vi "PicoScope2000aExampleBlockMSO.vi"() -> ()   [LabVIEW 2010]
doc: "ps2000a API Block Capture example"
uses:
  shared/PicoBuffers.ctl
  <vilib>/Waveform/DWDTOps.llb/DWDT Analog to Digital.vi
  shared/Buffer and Transfer Settings.ctl
  shared/Acquisition Settings.ctl
  PicoScope2000aLib/PicoScope2000aAnalogChannelSettings.ctl
  PicoScope2000aLib/PicoScope2000aDigitalChannelSettings.ctl
panel:
  out "Properties Panel":T1 {"Max Total Capture Time Available (sec)" format="%.3p"; "Sample Frequency" format="%.3p"; "Sample Internal" format="%.3p"; "Max Samples Available" format="%.3p"; "Total Capture Time (sec)" format="%.3p"}
  in  "Port 0 Settings":T2={"Enabled"=FALSE, "Logic Level"=9830} {"Logic Level" items=["1.5V TTL"=9830, "2.5V CMOS"=16383]}
  in  "Channel A Settings":T3={"Enabled"=TRUE, "Coupling"=1, "Range"=6, "Analogue Offset"=0.0} {"Analogue Offset" format="%#_6p"; "Range" items=["20 mV"=1, "50 mV"=2, "100 mV"=3, "200 mV"=4, "500 mV"=5, "1 V"=6, "2 V"=7, "5 V"=8, "10 V"=9, "20 V"=10]; "Coupling" items=["AC", "DC"]}
  out "Device Info":T4={"Driver Version"="2.1.104.3324", "USB Version"="2.0", "Hardware"="1", "Variant"="2206A", "Batch and Serial"="CV676/049", "Cal Date"="19Sep17", "Kernel Version"="1.0", "Digital HW Version"="1", "Analogue HW Version"="1", "Firmware 1"="1.3.3.0", "Firmware 2"="0.5.47.0", "MSO"=FALSE, "Number of Channels"=2}
  out "overflow":i16 format="%06b"
  in  "Apply Settings":bool
  in  "Trigger Settings":T5={"Trigger Enabled"=FALSE, "Trigger Source"=enum."Channel A", "Trigger Threshold (volts)"=0.0, "Trigger Direction"=2, "Trigger Delay (samples)"=0, "Auto Trigger Time (ms)"=1000} {"Trigger Direction" items=["Rising"=2, "Falling"=3]}
  out "error out":errorcluster
  in  "Data file":path=path "PicoScope2000aExampleBlock ChA Data"
  in  "Buffer and Transfer Settings":T6={"startIndex"=0, "Samples"=32000, "Down Sample Ratio"=1, "Down-Sample Mode"=0} {"Down-Sample Mode" items=["RAW none"=2147483648, "None"=0, "Aggregate"=1, "Decimate"=2, "Average"=4]; "Down Sample Ratio" step=1; "Samples" format="%_6p"}
  in  "Acquisition Settings":T7={"preTriggerSamples"=0, "postTriggerSamples"=32000, "timebase"=5} {"postTriggerSamples" format="%_6p"; "preTriggerSamples" format="%_6p"}
  out "Port 0":digitalwaveform(graph)={"t0"=timestamp(0 s since 1904-01-01), "dt"=8e-09, "Y"={"transitions"=[], "data"=[]}}
  in  "stop":bool
  out "Analog Channels":cluster{i32, sgl, "Data":dbl[]}[](graph)
  in  "Serial Number":string
  in  "Use Serial Number":bool
  in  "error in (no error)":errorcluster
  # "Bit 0 = ChA"
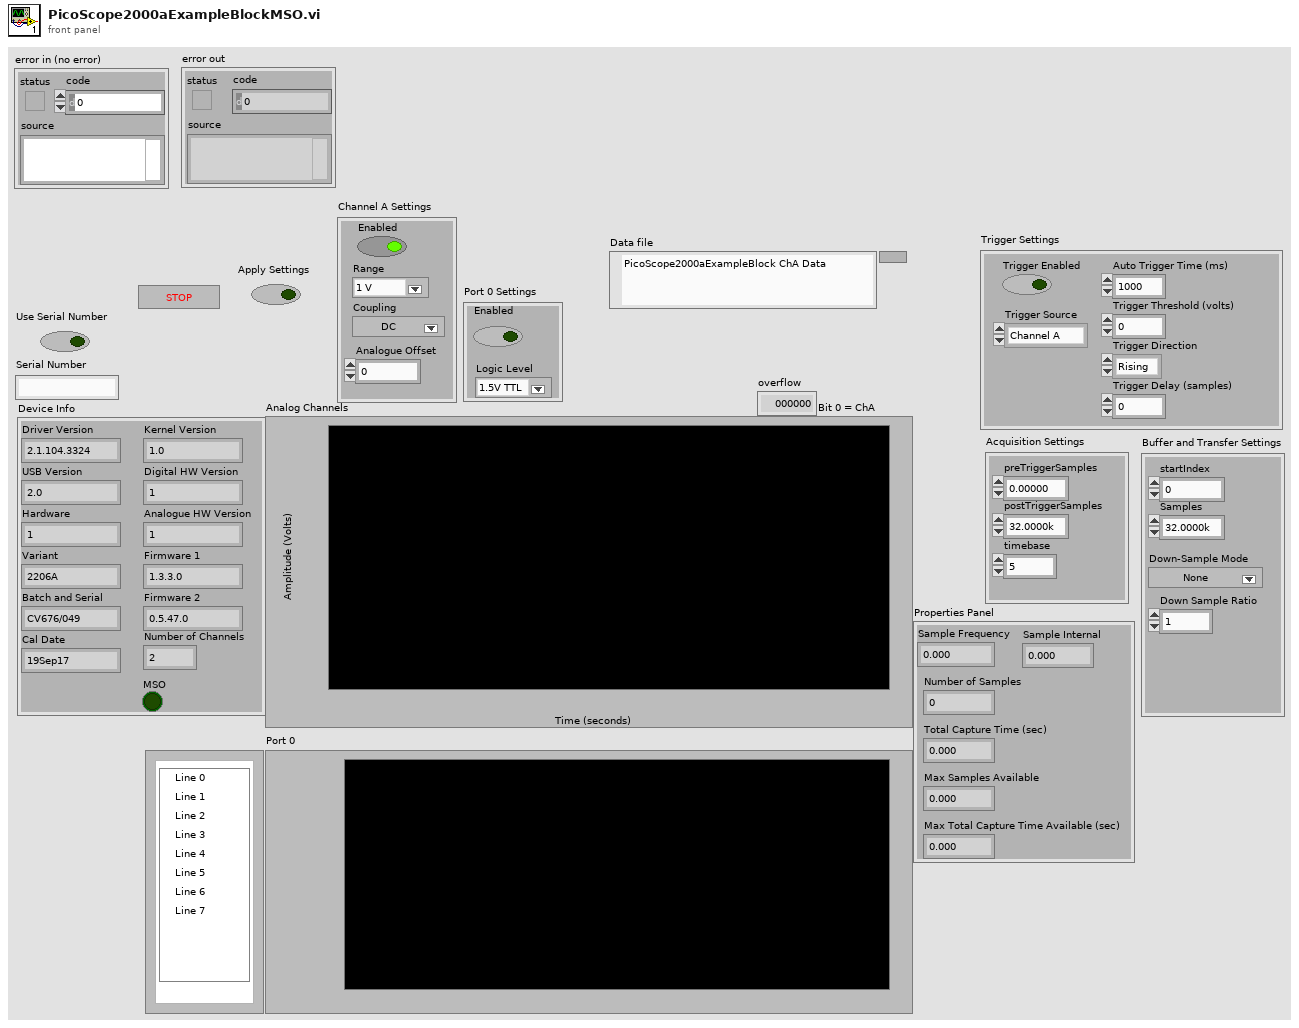
[diagram p1: front panel]
types:
  T1 = cluster{"Sample Frequency":sgl, "Sample Internal":sgl, "Max Samples Available":i32, "Number of Samples":u32, "Total Capture Time (sec) ":sgl, "Max Total Capture Time Available (sec)":sgl}
  T2 = typedef "PicoScope2000aDigitalChannelSettings.ctl" = cluster{"Enabled":bool, "Logic Level":i16}
  T3 = typedef "PicoScope2000aAnalogChannelSettings.ctl" = cluster{"Enabled":bool, "Coupling":i16, "Range":u16, "Analogue Offset":sgl}
  T4 = cluster{"Driver Version":string, "USB Version":string, "Hardware":string, "Variant":string, "Batch and Serial":string, "Cal Date":string, "Kernel Version":string, "Digital HW Version":string, "Analogue HW Version":string, "Firmware 1":string, "Firmware 2":string, "MSO":bool, "Number of Channels":i16}
  T5 = cluster{"Trigger Enabled":bool, "Trigger Source":enum16{"Channel A", "Channel B", "Channel C", "Channel D", "Ext."}, "Trigger Threshold (volts)":dbl, "Trigger Direction":u16, "Trigger Delay (samples)":u32, "Auto Trigger Time (ms)":i16}
  T6 = typedef "Buffer and Transfer Settings.ctl" = cluster{"startIndex":u64, "Samples":u64, "Down Sample Ratio":u64, "Down-Sample Mode":u32}
  T7 = typedef "Acquisition Settings.ctl" = cluster{"preTriggerSamples":u64, "postTriggerSamples":u64, "timebase":u32}
  T8 = enum16{"open", "open or create", "create or replace", "create", "open (read-only)"}
  T9 = typedef "PicoBuffers.ctl" = cluster{"Max Buffer Pointers":u64[][][], "Min Buffer Pointers":u64[][][], "StreamingDataInfo":cluster{"Channel":u32, "Down-Sample Mode":u32, "PICO_DATA_TYPE":enum32{"PICO_INT8_T", "PICO_INT16_T", "PICO_INT32_T", "PICO_UINT32_T", "PICO_INT64_T", ""}, "Samples":i32, "bufferIndex":u64, "startIndex":i32, "overflow":i16}[][]}
  T10 = cluster{"Channel A Buffer":i16[], "Channel B Buffer":i16[], "Channel C Buffer":i16[], "Channel D Buffer":i16[], "Channel E Buffer":i16[], "Channel F Buffer":i16[], "Channel G Buffer":i16[], "Channel H Buffer":i16[], "Port 0 Buffer":i16[], "Port 1 Buffer":i16[]}[]
  T11 = cluster{"Channel A Buffer":i16[], "Channel B Buffer":i16[], "Channel C Buffer":i16[], "Channel D Buffer":i16[], "Channel E Buffer":i16[], "Channel F Buffer":i16[], "Channel G Buffer":i16[], "Channel H Buffer":i16[], "Port 0 Buffer":i16[], "Port 1 Buffer":i16[]}
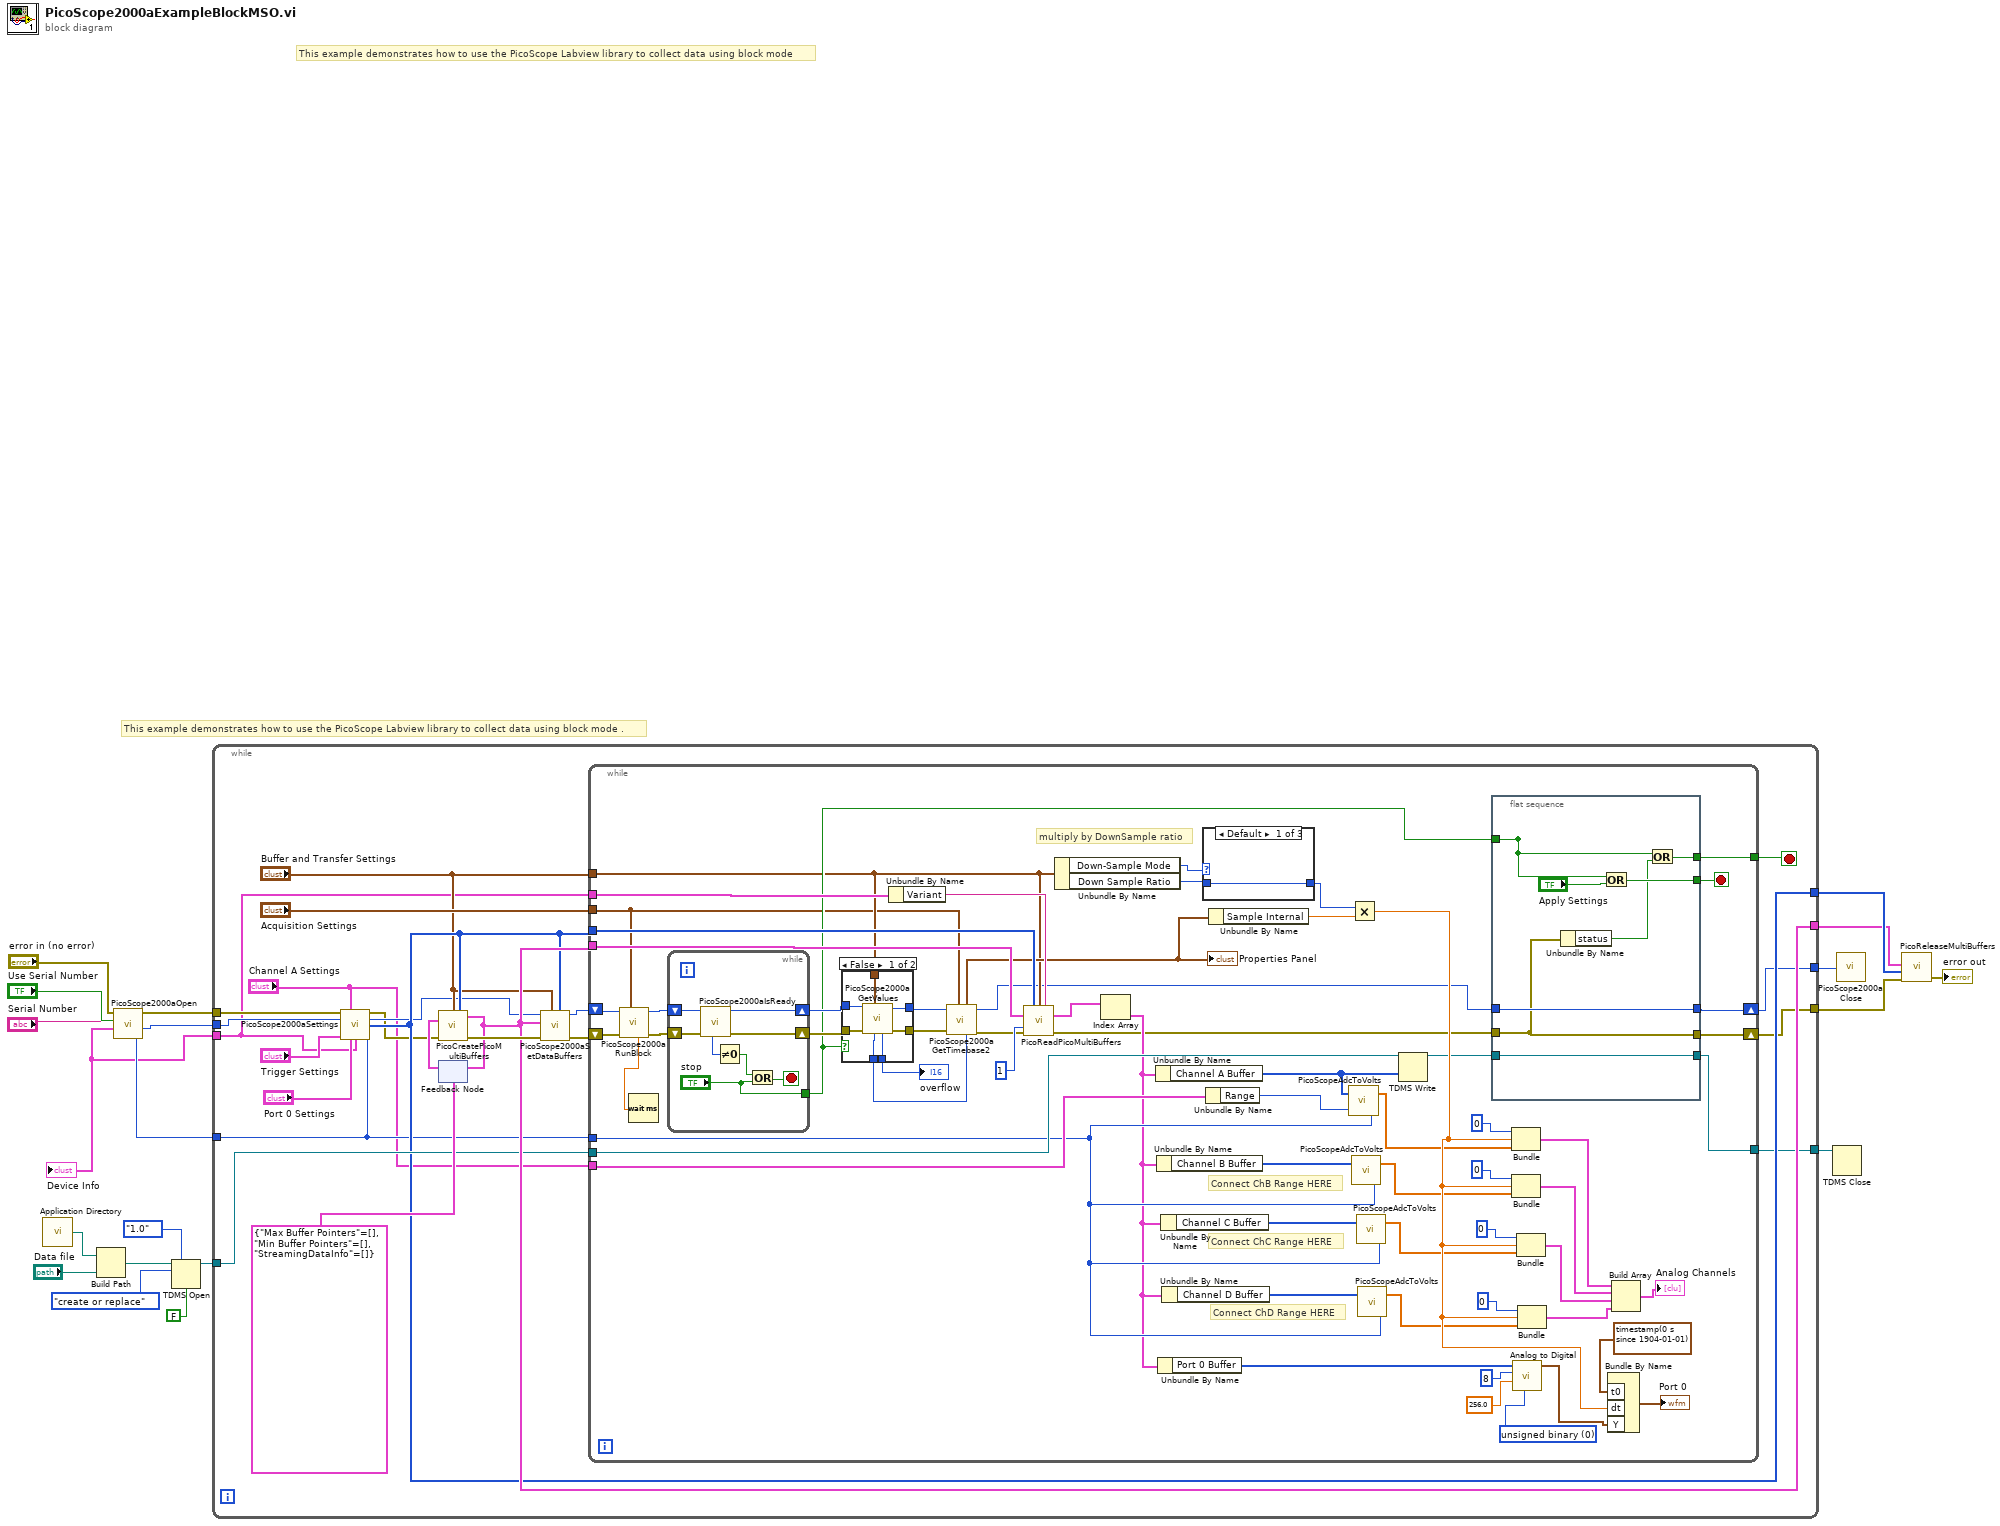
[diagram p0: block diagram]
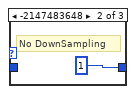
[diagram p3: hidden frame]
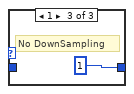
[diagram p4: hidden frame]
diagram:
  # "This example demonstrates how to use the PicoScope Labview library to collect data using block mode ."
  # "This example demonstrates how to use the PicoScope Labview library to collect data using block mode"
  n1 = call <vilib>:"Application Directory.vi"() -> ("Application Directory"=w12:path)
  n2 = Build Path(base path=w12, name or relative path="Data file") -> (appended path=w13:path)
  n3 = call "PicoScope2000aOpen.vi"("Serial Number"="Serial Number", "Use Serial Number"="Use Serial Number", "error in (no error)"="error in (no error)") -> ("Max Adc value"=w5:i16, "handle"=w20:i16, "error out"=w4:errorcluster, "Device Info"=w1:T4)  [unwired: 1 in]
  "Device Info" <- w1
  n4 = TDMS Open(6:FALSE ("disable buffering? (T)"), 7:enum16{"1.0", "2.0"}."1.0" ("file format version (2.0)"), 10:T8."create or replace" ("operation (0:open)"), 11:w13) -> (3:w10:refnum<k34>)  [unwired: 2 in, 1 out]
  n5 = while {
    tunnel: w20 -> [w38]
    tunnel: w5 -> [w33]
    tunnel: [w35] -> w19
    tunnel: [w40] -> w18
    tunnel: [w31] -> w11
    tunnel: w10 -> [w39]
    tunnel: w1 -> [w21]
    tunnel: w4 -> [w37]
    tunnel: [w32] -> w3
    tunnel: [w29] -> w2
    stop <- w30 stop-if-true
    n6 = call "PicoScope2000aSettings.vi"("error in"=w37, "Channel A Settings"="Channel A Settings", "handle in"=w38, "Trigger Settings"="Trigger Settings", "Port 0 Settings"="Port 0 Settings", "Device Info"=w21, "Max_adc"=w33) -> ("error out"=w24:errorcluster, "handle out"=w25:i16, "Enabled Array"=w35:i16[])  [unwired: 6 in]
    n7 = feedback #1(T9 {"Max Buffer Pointers"=[], "Min Buffer Pointers"=[], "StreamingDataInfo"=[]} ("Data Pointers")) -> (w42:T9)
    n8 = call "PicoCreatePicoMultiBuffers.vi"("Buffer and Transfer Settings"="Buffer and Transfer Settings", "enabled array"=w35, "Data Pointers In"=w42, "error in (no error)"=w24) -> ("Data Pointers"=w40:T9, "error out"=w41:errorcluster)  [unwired: 10 in]
    n9 = feedback-in #1(w40) -> ()
    n10 = call "PicoScope2000aSetDataBuffers.vi"("enabled array"=w35, "Buffer and Transfer Settings"="Buffer and Transfer Settings", "error in (no error)"=w41, "Data Pointers In"=w40, "handle in"=w25) -> ("error out"=w28:errorcluster, "handle out"=w27:i16)  [unwired: 5 in]
    n11 = while {
      tunnel: w40 -> [w107]
      tunnel: "Buffer and Transfer Settings" -> [w49]
      tunnel: w35 -> [w98]
      tunnel: "Channel A Settings" -> [w97]
      tunnel: "Acquisition Settings" -> [w48]
      tunnel: w33 -> [w96]
      tunnel: w21 -> [w93]
      tunnel: [w61] -> w30
      shift-right: [w65] -> w32
      shift-left: w28 -> [w55]
      shift-right: [w59] -> w29
      shift-left: w27 -> [w56]
      tunnel: w39 -> [w106]
      tunnel: [w63] -> w31
      stop <- w60 stop-if-true
      w82 = u16 0 items=["unsigned binary", "offset binary", "2's complement"] ("data format (offset binary)")
      # "Connect ChB Range HERE"
      # "Connect ChD Range HERE"
      # "Connect ChC Range HERE"
      # "multiply by DownSample ratio"
      n12 = call "PicoScope2000aRunBlock.vi"("Acquisition Settings"=w48, "error in (no error)"=w55, "handle in"=w56) -> ("error out"=w100:errorcluster, "handle out"=w99:i16, "timeIndisposedMs"=w50:dbl)  [unwired: 5 in, 1 out]
      n13 = Wait (ms)(milliseconds to wait=w50) -> ()  [unwired: 1 out]
      n14 = while {
        shift-right: [w131] -> w57
        shift-left: w100 -> [w132]
        shift-right: [w130] -> w58
        shift-left: w99 -> [w129]
        tunnel: ["stop"] -> w54
        stop <- w126 stop-if-true
        n15 = call "PicoScope2000aIsReady.vi"("error in (no error)"=w132, "handle in"=w129) -> ("error out"=w131:errorcluster, "handle out"=w130:i16, "ready"=w128:i16)  [unwired: 7 in]
        n16 = Not Equal To 0?(x=w128) -> (x != 0?=w127:bool)
        n17 = Or(x=w127, y="stop") -> (x .or. y?=w126:bool)
      }
      n18 = case shown="False" w54 {
        tunnel: w57 -> [w114 w115]
        tunnel: w58 -> [w113 w116]
        tunnel: [w112 w116] -> w46
        tunnel: [w111 w115] -> w47
        tunnel: w49 -> [w110 _]
        tunnel: [w109 _] -> w53
        tunnel: [w108 _] -> w52
        frame False {
          n19 = call "PicoScope2000aGetValues.vi"("Buffer and Transfer Settings"=w110, "error in (no error)"=w114, "handle in"=w113) -> ("error out"=w111:errorcluster, "handle out"=w112:i16, "overflow"=w109:i16, "noOfSamples"=w108:u64)  [unwired: 5 in]
        }
        frame True {
        }
      }
      "overflow" <- w53
      n20 = Unbundle By Name(w93) -> ("Variant"=w94:string)
      n21 = call "PicoScope2000aGetTimebase2.vi"("Number of Samples"=w52, "Acquisition Settings"=w48, "error in (no error)"=w47, "handle in"=w46) -> ("error out"=w45:errorcluster, "handle out"=w44:i16, "Properties Panel"=w51:T1)  [unwired: 5 in]
      "Properties Panel" <- w51
      n22 = call "PicoReadPicoMultiBuffers.vi"("enabled array"=w98, "Buffer and Transfer Settings"=w49, "Variant"=w94, "Data Pointers"=w107, "No of Buffers"=1, "error in (no error)"=w45) -> ("MultiBuffers (Max or non-aggregated)"=w105:T10, "error out"=w62:errorcluster)  [unwired: 7 in, 1 out]
      n23 = Unbundle By Name(w49) -> ("Down-Sample Mode"=w103:u32, "Down Sample Ratio"=w104:u64)
      n24 = Index Array(array=w105) -> (element=w66:T11)  [unwired: 1 in]
      n25 = Unbundle By Name(w66) -> ("Channel A Buffer"=w75:i16[])
      n26 = Unbundle By Name(w66) -> ("Channel B Buffer"=w88:i16[])
      n27 = Unbundle By Name(w66) -> ("Port 0 Buffer"=w80:i16[])
      n28 = Unbundle By Name(w66) -> ("Channel C Buffer"=w73:i16[])
      n29 = Unbundle By Name(w66) -> ("Channel D Buffer"=w69:i16[])
      n30 = case shown="Default" w103 {
        tunnel: [w133 u64 1 ("Down Sample Ratio") u64 1 ("Down Sample Ratio")] -> w101
        tunnel: w104 -> [w133 _ _]
        frame Default {
        }
        frame -2147483648 {
          # "No DownSampling"
        }
        frame 1 {
          # "No DownSampling"
        }
      }
      n31 = Unbundle By Name(w97) -> ("Range"=w90:u16)
      n32 = Unbundle By Name(w51) -> ("Sample Internal"=w95:sgl)
      n33 = call "PicoScopeAdcToVolts.vi"("Max_adc"=w96, "Range Index"=w90, "Data"=w75) -> ("Data"=w76:dbl[])
      n34 = Multiply(x=w101, y=w95) -> (x*y=w102:sgl)
      n35 = call "PicoScopeAdcToVolts.vi"("Max_adc"=w96, "Data"=w88) -> ("Data"=w87:dbl[])  [unwired: 1 in]
      n36 = call "PicoScopeAdcToVolts.vi"("Max_adc"=w96, "Data"=w73) -> ("Data"=w72:dbl[])  [unwired: 1 in]
      n37 = call "PicoScopeAdcToVolts.vi"("Max_adc"=w96, "Data"=w69) -> ("Data"=w68:dbl[])  [unwired: 1 in]
      n38 = TDMS Write(0:w106, 9:w75) -> (4:w64:refnum<k34>)  [unwired: 4 in, 3 out]
      n39 = flat-sequence {
        tunnel: [w124] -> w60
        tunnel: [w117] -> _
        tunnel: [w121] -> w61
        tunnel: w44 -> [w120]
        tunnel: [w120] -> w59
        tunnel: w62 -> [w119]
        tunnel: [w119] -> w65
        tunnel: [w118] -> w63
        tunnel: w64 -> [w118]
        tunnel: w54 -> [w117]
        frame #0 {
          n40 = Unbundle By Name(w119) -> ("status"=w122:bool)
          n41 = Or(x=w117, y="Apply Settings") -> (x .or. y?=w124:bool)
          n42 = Or(x=w117, y=w122) -> (x .or. y?=w121:bool)
        }
      }
      n43 = Bundle(0, w102, "Data"=w76) -> (w86:cluster{i32, sgl, "Data":dbl[]})  [unwired: 1 in]
      n44 = Bundle(0, w102, "Data"=w87) -> (w85:cluster{i32, sgl, "Data":dbl[]})  [unwired: 1 in]
      n45 = call-poly <vilib>:"Analog to Digital.vi"("data format (offset binary)"=w82, "full-scale range (pk-pk)"=256.0, "resolution (16 bit)"=8, "analog waveform"=w80) -> ("digital waveform"=w77:digitalwaveform)  [unwired: 4 in, 3 out]
      n46 = Bundle(0, w102, "Data"=w72) -> (w71:cluster{i32, sgl, "Data":dbl[]})  [unwired: 1 in]
      n47 = Bundle(0, w102, "Data"=w68) -> (w67:cluster{i32, sgl, "Data":dbl[]})  [unwired: 1 in]
      n48 = Bundle By Name("t0"=timestamp(0 s since 1904-01-01), "dt"=w102, "Y"=w77) -> (→"Port 0":digitalwaveform)  [unwired: 1 in]
      n49 = Build Array(w86, w85, w71, w67) -> (→"Analog Channels":cluster{i32, sgl, "Data":dbl[]}[])
    }
  }
  n50 = TDMS Close(11:w11) -> ()  [unwired: 1 in, 2 out]
  n51 = call "PicoScope2000aClose.vi"("handle"=w2) -> ()
  n52 = call "PicoReleaseMultiBuffers.vi"("error in (no error)"=w3, "Enabled array"=w19, "Data Pointers"=w18) -> ("error out"=→"error out":errorcluster)  [unwired: 8 in]
